vi "optical_low_level_get_image2.vi"() -> ()   [LabVIEW 2025]
uses:
  <vilib>/vision/driver/IMAQdx.llb/IMAQdx Buffer Number Mode.ctl
  <vilib>/vision/driver/IMAQdx.llb/IMAQdx Acquisition Mode.ctl
  <vilib>/vision/driver/NI_Vision_Acquisition_Software.lvlib
panel:
  in  "Buffer Number Mode (Next)":T1
  out "Image":T2(plugin-control)
  out "error out":errorcluster
  out "Times between Frames":u32
  in  "Output Folder":path
  in  "Stop":bool
  in  "Camera Name":refnum<k21> caption="IMAQdx Session"
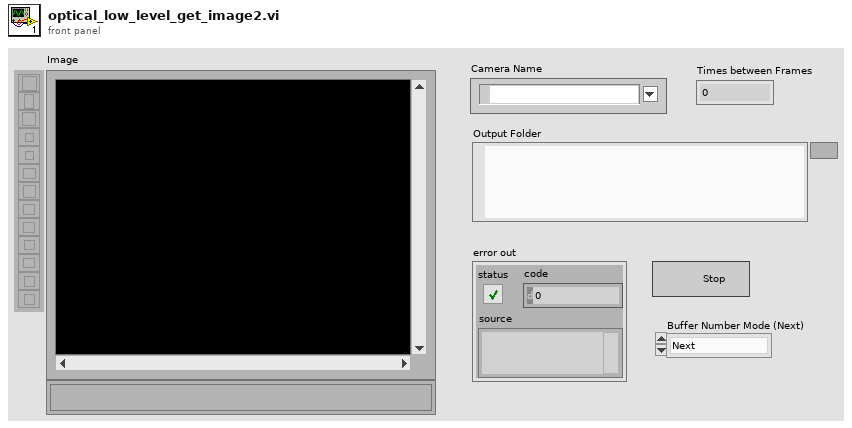
[diagram p1: front panel]
types:
  T1 = typedef "NI_Vision_Acquisition_Software.lvlib/IMAQdx Buffer Number Mode.ctl" = enum32{"Next", "Last", "Buffer Number", "Every", "Last New"}
  T2 = typedef "IMAQ Image.ctl" = refnum<image>
  T3 = typedef "Image Type" = u32
  T4 = typedef "NI_Vision_Acquisition_Software.lvlib/IMAQdx Acquisition Mode.ctl" = enum32{"One Shot", "Continuous"}
  T5 = typedef "IMAQdx.ctl" = refnum<k21>
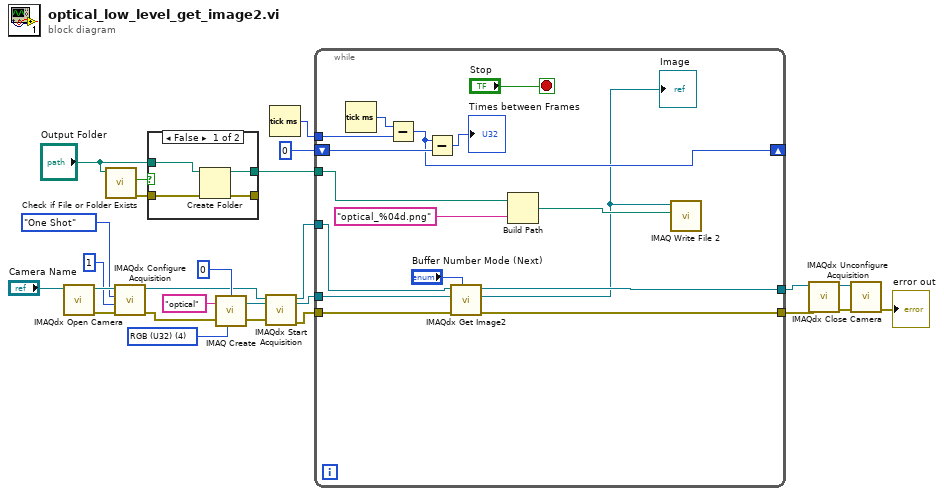
[diagram p0: block diagram]
diagram:
  w10 = T3 4 items=["Grayscale (U8)", "Grayscale (I16)", "Grayscale (SGL)", "Complex (CSG)", "RGB (U32)", "HSL (U32)", "RGB (U64)", "Grayscale (U16)"] ("Image Type")
  n1 = call <vilib>:"IMAQdx Open Camera.vi"("Session In"="Camera Name") -> ("error out"=w18:errorcluster, "Session Out"=w19:T5)  [unwired: 9 in]
  n2 = call <vilib>:"Check if File or Folder Exists.vi"("path"="Output Folder") -> ("error out"=w23:errorcluster, "file or folder exists?"=w25:bool)  [unwired: 8 in, 1 out]
  n3 = call <vilib>:"IMAQdx Configure Acquisition.vi"("error in"=w18, "Number of Buffers"=u32 1, "Continuous?"=IMAQdx_Acquisition_Mode."One Shot", "Session In"=w19) -> ("error out"=w12:errorcluster, "Session Out"=w3:T5)  [unwired: 6 in]
  n4 = case shown="False" w25 {
    tunnel: "Output Folder" -> [w29 w31]
    tunnel: [w28 w31] -> w22
    tunnel: w23 -> [w27 w30]
    tunnel: [w26 w30] -> _
    frame False {
      n5 = Create Folder(path (use dialog)=w29, error in=w27) -> (created path=w28:path, error out=w26:errorcluster)  [unwired: 1 in, 1 out]
    }
    frame True {
    }
  }
  n6 = call "IMAQ Create"("Border Size"=0, "Image Name"="optical", "Image Type"=w10, "error in (no error)"=w12) -> ("New Image"=w13:T2, "error out"=w4:errorcluster)  [unwired: 1 in]
  n7 = call <vilib>:"IMAQdx Start Acquisition.vi"("error in"=w4, "Session In"=w3) -> ("error out"=w2:errorcluster, "Session Out"=w1:T5)  [unwired: 8 in]
  n8 = Tick Count (ms)() -> (millisecond timer value=w21:u32)
  n9 = while {
    tunnel: w22 -> [w47]
    tunnel: w21 -> [w45]
    shift-right: [w42] -> _
    shift-left: u32 0 -> [w43]
    tunnel: [w37] -> w8
    tunnel: [w35] -> w6
    tunnel: w13 -> [w39]
    tunnel: w2 -> [w33]
    tunnel: w1 -> [w32]
    stop <- "Stop" stop-if-true
    n10 = Tick Count (ms)() -> (millisecond timer value=w46:u32)
    n11 = Subtract(x=w46, y=w45) -> (x-y=w42:u32)
    n12 = Subtract(x=w42, y=w43) -> (x-y=→"Times between Frames":u32)
    n13 = call <vilib>:"IMAQdx Get Image2.vi"("Buffer Number Mode (Next)"="Buffer Number Mode (Next)", "error in"=w33, "Image In"=w39, "Session In"=w32) -> ("error out"=w35:errorcluster, "Image Out"=w36:T2, "Session Out"=w37:T5)  [unwired: 4 in, 1 out]
    "Image" <- w36
    n14 = Build Path(base path=w47, name or relative path="optical_%04d.png" ("format string")) -> (appended path=w41:path)
    n15 = call-poly "IMAQ Write File 2"("File Path"=w41, "Image"=w36) -> ()  [unwired: 8 in, 2 out]
  }
  n16 = call <vilib>:"IMAQdx Unconfigure Acquisition.vi"("error in"=w6, "Session In"=w8) -> ("error out"=w5:errorcluster, "Session Out"=w7:T5)  [unwired: 8 in]
  n17 = call <vilib>:"IMAQdx Close Camera.vi"("error in"=w5, "Session In"=w7) -> ("error out"=→"error out":errorcluster)  [unwired: 9 in]
